vi "avaiable tag menu action.vi"(6 "Call Back VI":T1, 8 "channel":refnum<class "TBM channel.lvclass">, 9 "selected tag":refnum<class "tag descriptor.lvclass">, 10 "action":T2, 11 "object ref":T3) -> (0 "error out":errorcluster, 2 "update?":bool)   [LabVIEW 2014, in "Table Manager.lvlib"]
uses:
  Table Manager.lvlib
  Table Manager/object ref.ctl
  Configuration Editor/Classes/Engine Parent/Engine Parent Editor Node.lvclass
  Configuration Editor/Classes/Module editor node/module editor node.lvclass
  <vilib>/NI/Tag Bus/tag/tag descriptor.lvclass
  <vilib>/NI/Tag Bus Module Framework/channel/TBM channel.lvclass
  dialog output action.ctl
  Table Manager/Call Back Ref Type Def.ctl
  <vilib>/NI/Configuration Framework/serializable configuration/NISE_CEF_serializable configuration.lvclass/NISE_CEF_serializable configuration.ctl
  Table Manager/Cell Change.ctl
  <vilib>/Utility/LVClass/Get LV Class Name.vi
  <vilib>/NI/Configuration Framework/error generator/NISE_error generator.vi
  Configuration Editor/Classes/Module editor node/Read Module Configuration.vi
  <vilib>/NI/Tag Bus Module Framework/module configuration/TBM module configuration.lvclass
  <vilib>/NI/Module Execution Interface/Engine Configuration/engine configuration.lvclass
  <vilib>/NI/Configuration Framework/serializable configuration/NISE_CEF_serializable configuration.lvclass
  control module/editor node/control module editor.lvclass
  Table Manager/Table Manager.lvclass
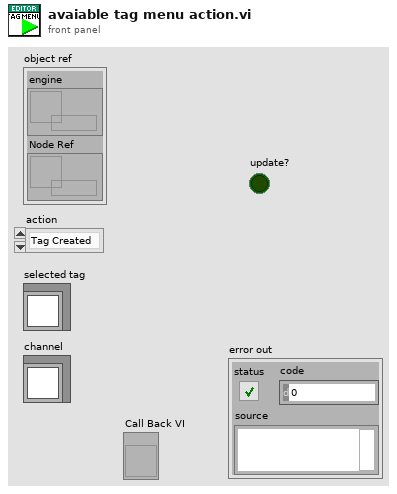
[diagram p1: front panel]
types:
  T1 = typedef "Table Manager.lvlib/Table Manager.lvclass/Call Back Ref Type Def.ctl" = refnum<vi>
  T2 = typedef "Table Manager.lvlib/dialog output action.ctl" = enum16{"Tag Created", "Tag Selected", "Set Default", "disconnect"}
  T3 = typedef "Table Manager.lvlib/Table Manager.lvclass/object ref.ctl" = cluster{"engine":refnum<data-value>, "Node Ref":refnum<data-value>}
  T4 = typedef "Table Manager.lvlib/Cell Change.ctl" = cluster{"row":i32, "col":i32, "old value":string, "new value":string}
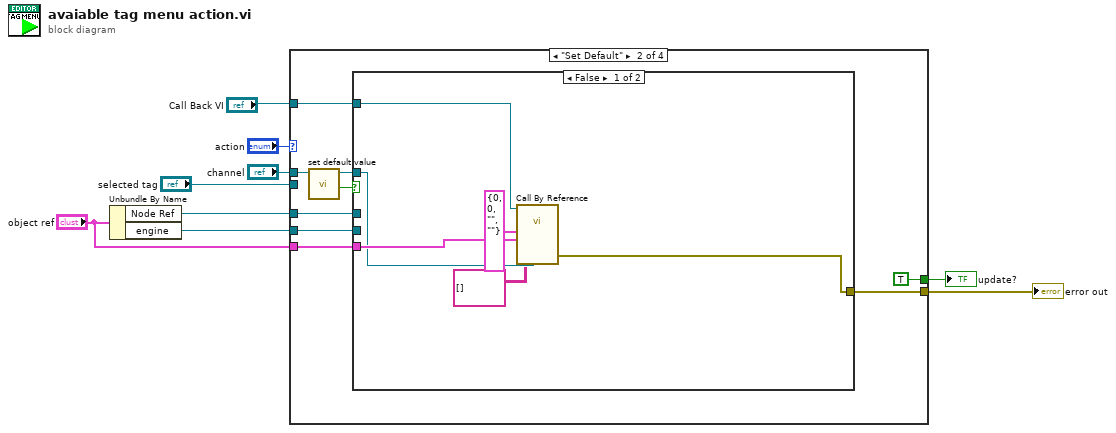
[diagram p0: block diagram]
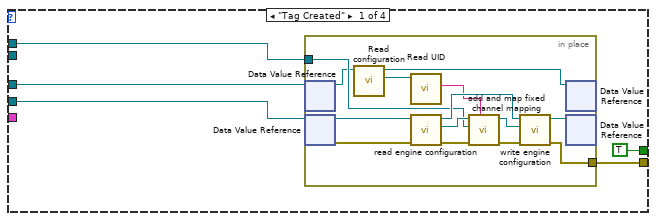
[diagram p2: hidden frame]
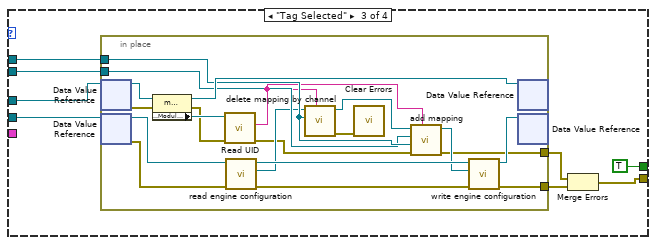
[diagram p4: hidden frame]
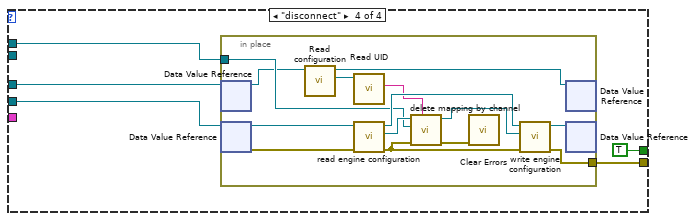
[diagram p5: hidden frame]
diagram:
  n1 = Unbundle By Name("object ref") -> ("Node Ref"=w8:refnum<data-value>, "engine"=w9:refnum<data-value>)
  n2 = case shown="\"Set Default\"" "action" {
    tunnel: "channel" -> [w14 w35 w50 w76]
    tunnel: "selected tag" -> [_ _ w46 _]
    tunnel: [w11 w37 w51 w74] -> w7
    tunnel: w8 -> [w12 w36 w45 w73]
    tunnel: w9 -> [w13 w32 w49 w75]
    tunnel: [TRUE ("update?") TRUE ("update?") TRUE ("update?") TRUE ("update?")] -> w3
    tunnel: "Call Back VI" -> [_ w30 _ _]
    tunnel: "object ref" -> [_ w29 _ _]
    frame "Tag Created" {
      n3 = in-place {
        in-place-border: [w25] -> w11
        in-place-border: w14 -> [w21]
        n4 = in-place-dvr #1(w12) -> (w18:refnum<class "module editor node.lvclass">)  [unwired: 1 out]
        n5 = in-place-dvr #2(w13) -> (w27:refnum<class "Engine Parent Editor Node.lvclass">, w28:errorcluster)
        n6 = call-dynamic "Read configuration.vi"("NISE_CEF_serializable node in"=w18) -> ("configuration"=w16:refnum<class "NISE_CEF_serializable configuration.lvclass">, "NISE_CEF_serializable node out"=w17:refnum<class "module editor node.lvclass">)  [unwired: 8 in, 1 out]
        n7 = call <vilib>:"Read UID.vi"("configuration in"=w16) -> ("instance id"=w15:string)  [unwired: 8 in, 2 out]
        n8 = call "read engine configuration.vi"("error in"=w28, "Engine Parent Editor Node in"=w27) -> ("error out"=w20:errorcluster, "engine configuration"=w23:refnum<class "engine configuration.lvclass">, "Engine Parent Editor Node out"=w24:refnum<class "Engine Parent Editor Node.lvclass">)  [unwired: 7 in]
        n9 = call <vilib>:"add and map fixed channel mapping.vi"("module instance"=w15, "error in"=w20, "fixed channel"=w21, "engine configuration in"=w23) -> ("error out"=w19:errorcluster, "engine configuration out"=w22:refnum<class "engine configuration.lvclass">)  [unwired: 6 in]
        n10 = call "write engine configuration.vi"("error in"=w19, "engine configuration"=w22, "Engine Parent Editor Node in"=w24) -> ("error out"=w25:errorcluster, "Engine Parent Editor Node out"=w26:refnum<class "Engine Parent Editor Node.lvclass">)  [unwired: 7 in]
        n11 = in-place-dvr #1(w17) -> ()  [unwired: 2 out]
        n12 = in-place-dvr #2(w26) -> ()  [unwired: 2 out]
      }
    }
    frame "Set Default" {
      n13 = call "set default value.vi"("tag"=w35) -> ("cancelled?"=w33:bool, "tag out"=w34:refnum<class "TBM channel.lvclass">)  [unwired: 9 in]
      n14 = case shown="False" w33 {
        tunnel: [w40 _] -> w37
        tunnel: w36 -> [_ _]
        tunnel: w34 -> [w41 _]
        tunnel: w32 -> [_ _]
        tunnel: w30 -> [w43 _]
        tunnel: w29 -> [w42 _]
        frame False {
          n15 = call-by-ref "?"(reference=w43, "Variant"=w41, "old values"=string[][] [], "object ref in"=w42, "Table Change"=T4 {"row"=0, "col"=0, "old value"="", "new value"=""}) -> ("error out"=w40:errorcluster)  [unwired: 8 in, 2 out]
        }
        frame True {
        }
      }
    }
    frame "Tag Selected" {
      n16 = in-place {
        in-place-border: [w61] -> w48
        in-place-border: w50 -> [w69]
        in-place-border: [w66] -> w47
        in-place-border: w46 -> [w60]
        n17 = in-place-dvr #3(w45) -> (w71:refnum<class "module editor node.lvclass">, w68:errorcluster)
        n18 = in-place-dvr #4(w49) -> (w64:refnum<class "Engine Parent Editor Node.lvclass">, w65:errorcluster)
        n19 = property class="module editor node"(reference=w71, error in=w68) -> (reference out=w70:refnum<class "module editor node.lvclass">, error out=w54:errorcluster, "Data Access:Module Configuration"=w56:refnum<class "TBM module configuration.lvclass">)
        n20 = call <vilib>:"Read UID.vi"("error in"=w54, "configuration in"=w56) -> ("error out"=w53:errorcluster, "instance id"=w57:string)  [unwired: 7 in, 1 out]
        n21 = call "read engine configuration.vi"("error in"=w65, "Engine Parent Editor Node in"=w64) -> ("error out"=w55:errorcluster, "engine configuration"=w59:refnum<class "engine configuration.lvclass">, "Engine Parent Editor Node out"=w63:refnum<class "Engine Parent Editor Node.lvclass">)  [unwired: 7 in]
        n22 = call <vilib>:"delete mapping by channel.vi"("owner ID"=w57, "channel"=w69, "engine configuration in"=w59) -> ("error out"=w52:errorcluster, "engine configuration out"=w58:refnum<class "engine configuration.lvclass">)  [unwired: 7 in]
        n23 = call <vilib>:"Clear Errors.vi"("error in (no error)"=w52) -> ()  [unwired: 5 in, 2 out]
        n24 = call-dynamic "add mapping.vi"("owner ID"=w57, "error in"=w53, "channel"=w69, "tag descriptor"=w60, "engine configuration"=w58) -> ("error out"=w61:errorcluster, "engine configuration out"=w62:refnum<class "engine configuration.lvclass">)  [unwired: 5 in]
        n25 = call "write engine configuration.vi"("error in"=w55, "engine configuration"=w62, "Engine Parent Editor Node in"=w63) -> ("error out"=w66:errorcluster, "Engine Parent Editor Node out"=w67:refnum<class "Engine Parent Editor Node.lvclass">)  [unwired: 7 in]
        n26 = in-place-dvr #3(w70) -> ()  [unwired: 2 out]
        n27 = in-place-dvr #4(w67) -> ()  [unwired: 2 out]
      }
      n28 = Merge Errors(w48, w47) -> (w51:errorcluster)
    }
    frame "disconnect" {
      n29 = in-place {
        in-place-border: w76 -> [w82]
        in-place-border: [w87] -> w74
        n30 = in-place-dvr #5(w73) -> (w77:refnum<class "module editor node.lvclass">)  [unwired: 1 out]
        n31 = in-place-dvr #6(w75) -> (w90:refnum<class "Engine Parent Editor Node.lvclass">, w89:errorcluster)
        n32 = call-dynamic "Read configuration.vi"("NISE_CEF_serializable node in"=w77) -> ("configuration"=w80:refnum<class "NISE_CEF_serializable configuration.lvclass">, "NISE_CEF_serializable node out"=w78:refnum<class "module editor node.lvclass">)  [unwired: 8 in, 1 out]
        n33 = call <vilib>:"Read UID.vi"("configuration in"=w80) -> ("instance id"=w79:string)  [unwired: 8 in, 2 out]
        n34 = call "read engine configuration.vi"("error in"=w89, "Engine Parent Editor Node in"=w90) -> ("error out"=w84:errorcluster, "engine configuration"=w85:refnum<class "engine configuration.lvclass">, "Engine Parent Editor Node out"=w86:refnum<class "Engine Parent Editor Node.lvclass">)  [unwired: 7 in]
        n35 = call <vilib>:"delete mapping by channel.vi"("owner ID"=w79, "error in"=w84, "channel"=w82, "engine configuration in"=w85) -> ("error out"=w81:errorcluster, "engine configuration out"=w83:refnum<class "engine configuration.lvclass">)  [unwired: 6 in]
        n36 = call <vilib>:"Clear Errors.vi"("error in (no error)"=w81) -> ()  [unwired: 5 in, 2 out]
        n37 = call "write engine configuration.vi"("error in"=w84, "engine configuration"=w83, "Engine Parent Editor Node in"=w86) -> ("error out"=w87:errorcluster, "Engine Parent Editor Node out"=w88:refnum<class "Engine Parent Editor Node.lvclass">)  [unwired: 7 in]
        n38 = in-place-dvr #5(w78) -> ()  [unwired: 2 out]
        n39 = in-place-dvr #6(w88) -> ()  [unwired: 2 out]
      }
    }
  }
  "error out" <- w7
  "update?" <- w3
